vi "Clear Mock.vi"(8 "error in (no error)":errorcluster, 11 "Mock In":refnum<class "LMock Mock.lvclass">) -> (0 "error out":errorcluster)   [LabVIEW 2020, in "LMock Mock.lvclass"]
doc: "Template method which should be overriden to clear anything which has been initialized during the lifecycle of the mock class. \nThis VI is called when the mock is verified, which marks the end of its lifecycle."
uses:
  LMock Mock.lvclass
  LMock Mock.lvclass/LMock Mock.ctl
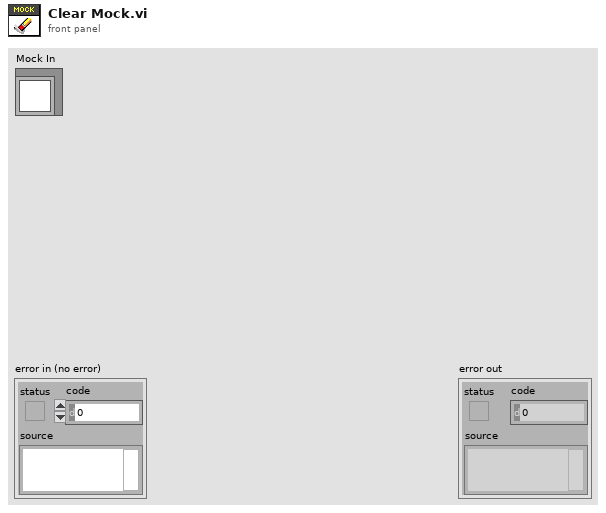
[diagram p1: front panel]
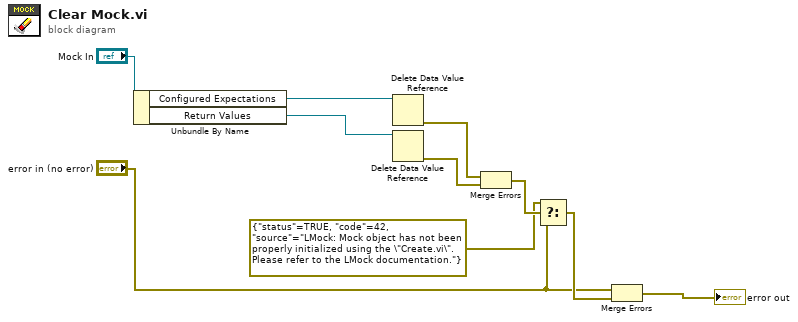
[diagram p0: block diagram]
diagram:
  n1 = Unbundle By Name("Mock In") -> ("Configured Expectations"=w9:refnum<data-value>, "Return Values"=w7:refnum<data-value>)
  n2 = Delete Data Value Reference(data value reference=w9) -> (error out=w8:errorcluster)  [unwired: 1 in, 1 out]
  n3 = Delete Data Value Reference(data value reference=w7) -> (error out=w6:errorcluster)  [unwired: 1 in, 1 out]
  n4 = Merge Errors(w8, w6) -> (w5:errorcluster)
  n5 = Select(t=errorcluster {"status"=TRUE, "code"=42, "source"="LMock: Mock object has not been properly initialized using the \"Create.vi\". Please refer to the LMock documentation."} ("f"), s=w5, f="error in (no error)") -> (s? t:f=w2:errorcluster)
  n6 = Merge Errors("error in (no error)", w2) -> (→"error out":errorcluster)
